vi "Handle Error.vi"(8 "error in (no error)":errorcluster caption="에러 입력(에러 없음)", 11 "TCP Socket 입력":refnum<class "TCP Socket.lvclass">) -> (0 "error out":errorcluster caption="에러 출력", 3 "TCP Socket 출력":refnum<class "TCP Socket.lvclass">)   [LabVIEW 2023, in "TCP Socket.lvclass"]
uses:
  TCP Socket.lvclass
  TCP Socket.lvclass/TCP Socket.ctl
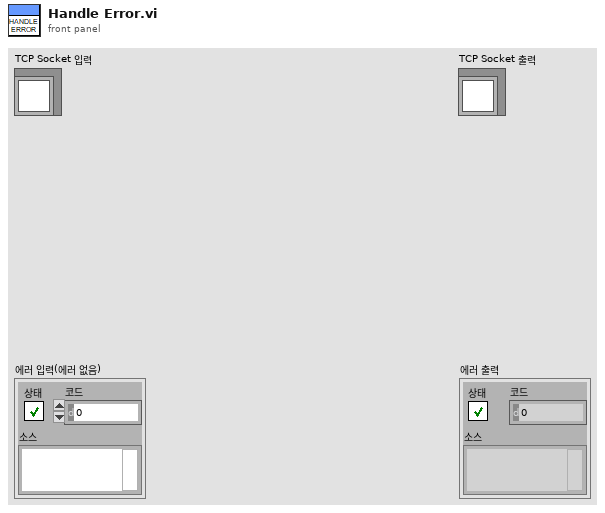
[diagram p1: front panel]
types:
  T1 = enum16{"big-endian, network order", "native, host order", "little-endian"}
  T2 = cluster{"Reader Q":refnum<queue>, "Writer Q":refnum<queue>}
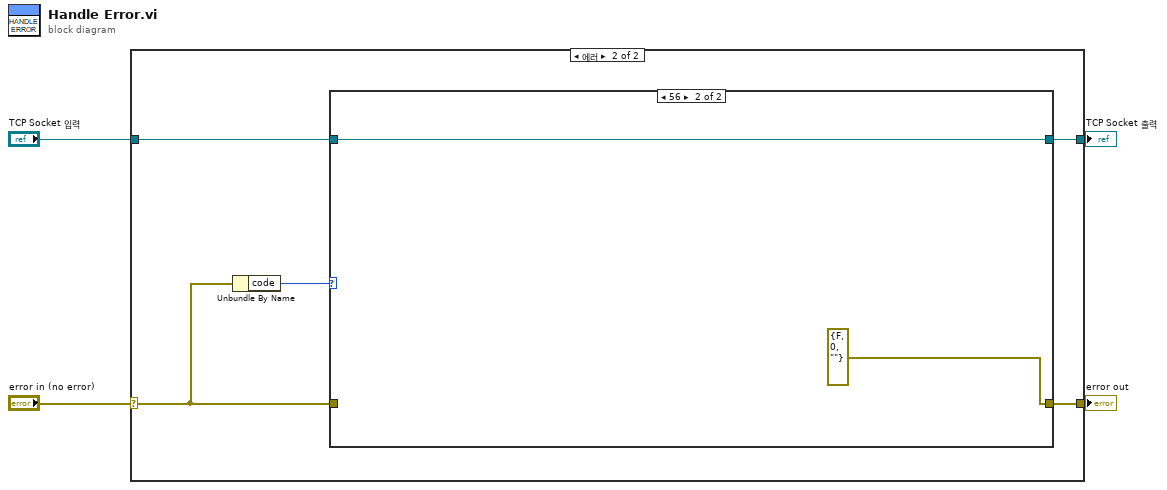
[diagram p0: block diagram]
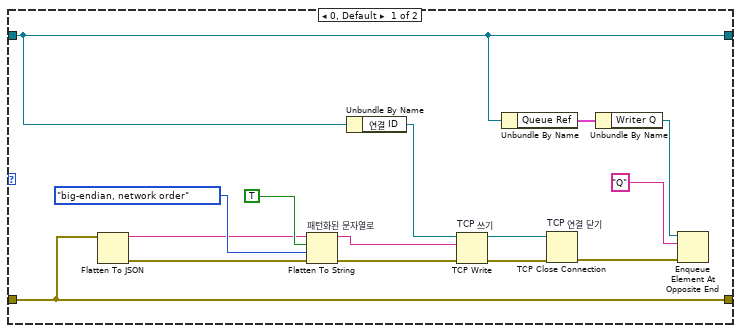
[diagram p3: hidden frame]
diagram:
  n1 = case shown="에러" "error in (no error)" {
    selector: "error in (no error)" -> [w5 w10]
    tunnel: [w5 w8] -> w3
    tunnel: [w6 w7] -> w1
    tunnel: "TCP Socket 입력" -> [w6 w9]
    frame No Error {
      # "경고가 전달되도록 에러 클러스터를\n\"에러 없음\" 케이스까지 연결합니다."
    }
    frame Error {
      n2 = Unbundle By Name(w10) -> ("code"=w11:i32)
      n3 = case shown="56" w11 {
        tunnel: w10 -> [w17 _]
        tunnel: w9 -> [w15 w28]
        tunnel: [w17 errorcluster {"status"=FALSE, "code"=0, "source"=""} ("error IO")] -> w8
        tunnel: [w15 w28] -> w7
        frame 0, Default {
          n4 = Flatten To JSON(anything=w17) -> (JSON string=w23:string, 11:w24:errorcluster)  [unwired: 2 in]
          n5 = Flatten To String "패턴화된 문자열로"(anything=w23, prepend array or string size? (T)=TRUE ("배열 또는 문자열 크기를 앞에 추가? (참)"), byte order (0:big-endian, network order)=T1."big-endian, network order" ("바이트 순서(0:big-endian, network order)"), error in (no error)=w24) -> (data string=w18:string, error out=w22:errorcluster)  [unwired: 1 out]
          n6 = Unbundle By Name(w15) -> ("연결 ID"=w20:refnum<k5>)
          n7 = TCP Write "TCP 쓰기"(connection ID=w20, data in=w18, error in (no error)=w22) -> (connection ID out=w19:refnum<k5>, error out=w21:errorcluster)  [unwired: 1 in, 1 out]
          n8 = Unbundle By Name(w15) -> ("Queue Ref"=w14:T2)
          n9 = TCP Close Connection "TCP 연결 닫기"(connection ID=w19, error in (no error)=w21) -> (error out=w16:errorcluster)  [unwired: 1 in, 1 out]
          n10 = Unbundle By Name(w14) -> ("Writer Q"=w13:refnum<queue>)
          n11 = Enqueue Element At Opposite End(queue=w13, element="Q" ("원소"), error in (no error)=w16) -> ()  [unwired: 1 in, 3 out]
        }
        frame 56 {
        }
      }
    }
  }
  "error out" <- w3
  "TCP Socket 출력" <- w1
